vi "VIH - VI Doc Editor #2 - GenObject Properties - Write.vi"(8 "error in":errorcluster, 10 "Props":T1, 11 "Ctrl Refnum":refnum<vi>) -> (0 "error out":errorcluster, 3 "dup Ctrl Refnum":refnum<vi>)   [LabVIEW 2014]
doc: "::: VI Helpeks :::\nCopyright (c) 2000-2026 Konstantin Shifershteyn. All rights reserved."
panel:
  # "VI Helpeks\nCopyright (c) 2012-2026 Konstantin Shifershteyn"
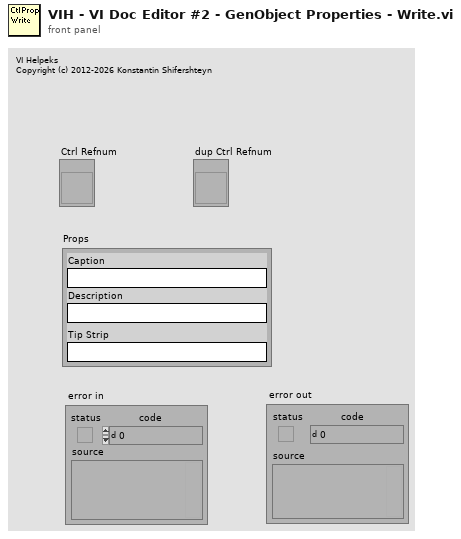
[diagram p1: front panel]
types:
  T1 = cluster{"Caption":string, "Description":string, "Tip Strip":string}
  T2 = cluster{"Has Caption":bool, "Caption":string, "Description":string, "Tip Strip":string}
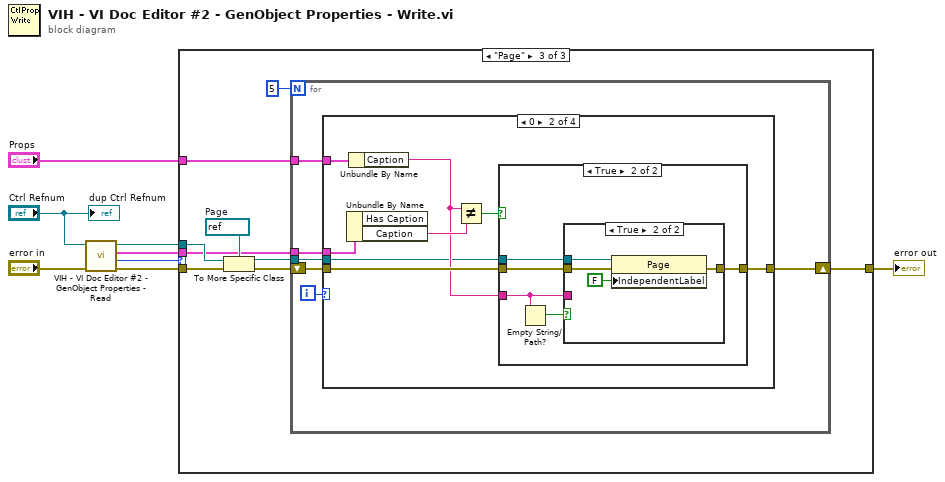
[diagram p0: block diagram]
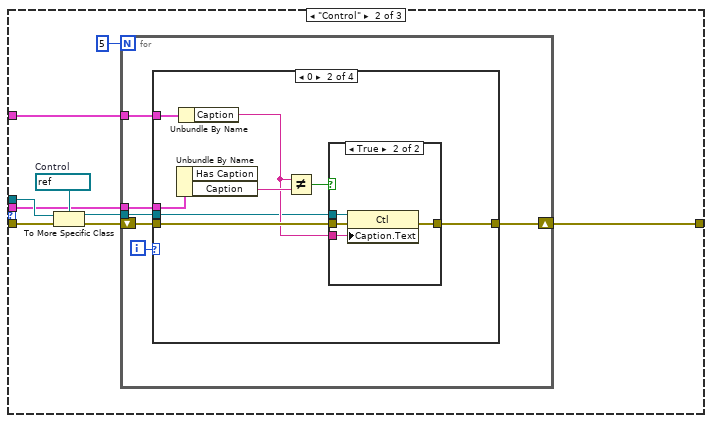
[diagram p3: hidden frame]
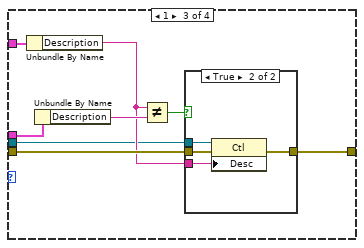
[diagram p6: hidden frame]
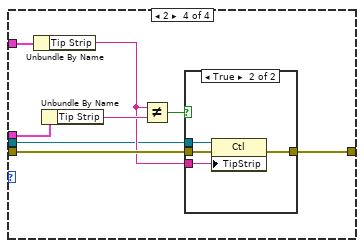
[diagram p8: hidden frame]
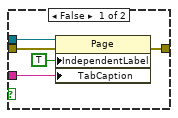
[diagram p12: hidden frame]
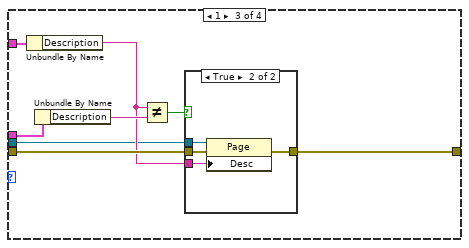
[diagram p13: hidden frame]
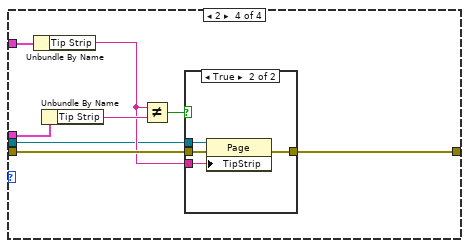
[diagram p15: hidden frame]
diagram:
  n1 = call "VIH - VI Doc Editor #2 - GenObject Properties - Read.vi"("error in"="error in", "Gen Refnum"="Ctrl Refnum") -> ("error out"=w3:errorcluster, "type"=w4:enum16{"<Invalid>", "Control", "Page"}, "Props"=w1:T2, "dup Gen Refnum"=w2:refnum<vi>)  [unwired: 6 in]
  n2 = case shown="\"Page\"" w4 {
    tunnel: "Props" -> [_ w17 w72]
    tunnel: [w9 w16 w71] -> w7
    tunnel: w3 -> [w9 w14 w69]
    tunnel: w2 -> [_ w12 w67]
    tunnel: w1 -> [_ w10 w65]
    frame "<Invalid>" {
    }
    frame "Control" {
      w15 = refnum<vi> refnum  # Control
      n3 = To More Specific Class(target class=w15, reference=w12, error in=w14) -> (specific class reference=w11:refnum<vi>, error out=w13:errorcluster)
      n4 = for {
        N: 5 -> [_]
        tunnel: w10 -> [w24]
        tunnel: w17 -> [w22]
        shift-right: [w20] -> w16
        shift-left: w13 -> [w21]
        tunnel: w11 -> [w19]
        i -> [w23]
        n5 = case shown="0" w23 {
          tunnel: w24 -> [_ w33 w46 w59]
          tunnel: w22 -> [_ w32 w45 w58]
          tunnel: w21 -> [w25 w31 w44 w57]
          tunnel: [w25 w30 w43 w56] -> w20
          tunnel: w19 -> [_ w26 w39 w52]
          frame Default {
          }
          frame 0 {
            n6 = Unbundle By Name(w33) -> ("Caption"=w29:string)  [unwired: 1 out]
            n7 = Unbundle By Name(w32) -> ("Caption"=w28:string)
            n8 = Not Equal?(x=w28, y=w29) -> (x != y?=w27:bool)
            n9 = case shown="True" w27 {
              tunnel: w31 -> [w34 w38]
              tunnel: [w34 w37] -> w30
              tunnel: w28 -> [_ w36]
              tunnel: w26 -> [_ w35]
              frame False {
              }
              frame True {
                n10 = property class="Ctl"(reference=w35, error in=w38, "Caption.Text"=w36) -> (error out=w37:errorcluster)  [unwired: 1 out]
              }
            }
          }
          frame 1 {
            n11 = Unbundle By Name(w45) -> ("Description"=w41:string)
            n12 = Unbundle By Name(w46) -> ("Description"=w42:string)
            n13 = Not Equal?(x=w41, y=w42) -> (x != y?=w40:bool)
            n14 = case shown="True" w40 {
              tunnel: w44 -> [w47 w51]
              tunnel: [w47 w50] -> w43
              tunnel: w41 -> [_ w49]
              tunnel: w39 -> [_ w48]
              frame False {
              }
              frame True {
                n15 = property class="Ctl"(reference=w48, error in=w51, "Desc"=w49) -> (error out=w50:errorcluster)  [unwired: 1 out]
              }
            }
          }
          frame 2 {
            n16 = Unbundle By Name(w58) -> ("Tip Strip"=w54:string)
            n17 = Unbundle By Name(w59) -> ("Tip Strip"=w55:string)
            n18 = Not Equal?(x=w54, y=w55) -> (x != y?=w53:bool)
            n19 = case shown="True" w53 {
              tunnel: w57 -> [w60 w64]
              tunnel: [w60 w63] -> w56
              tunnel: w54 -> [_ w62]
              tunnel: w52 -> [_ w61]
              frame False {
              }
              frame True {
                n20 = property class="Ctl"(reference=w61, error in=w64, "TipStrip"=w62) -> (error out=w63:errorcluster)  [unwired: 1 out]
              }
            }
          }
        }
      }
    }
    frame "Page" {
      w70 = refnum<vi> refnum  # Page
      n21 = To More Specific Class(target class=w70, reference=w67, error in=w69) -> (specific class reference=w66:refnum<vi>, error out=w68:errorcluster)
      n22 = for {
        N: 5 -> [_]
        tunnel: w65 -> [w79]
        tunnel: w72 -> [w77]
        shift-right: [w75] -> w71
        shift-left: w68 -> [w76]
        tunnel: w66 -> [w74]
        i -> [w78]
        n23 = case shown="0" w78 {
          tunnel: w79 -> [_ w88 w111 w124]
          tunnel: w77 -> [_ w87 w110 w123]
          tunnel: w76 -> [w80 w86 w109 w122]
          tunnel: [w80 w85 w108 w121] -> w75
          tunnel: w74 -> [_ w81 w104 w117]
          frame Default {
          }
          frame 0 {
            n24 = Unbundle By Name(w88) -> ("Caption"=w84:string)  [unwired: 1 out]
            n25 = Unbundle By Name(w87) -> ("Caption"=w83:string)
            n26 = Not Equal?(x=w83, y=w84) -> (x != y?=w82:bool)
            n27 = case shown="True" w82 {
              tunnel: w86 -> [w89 w94]
              tunnel: [w89 w93] -> w85
              tunnel: w83 -> [_ w90]
              tunnel: w81 -> [_ w92]
              frame False {
              }
              frame True {
                n28 = Empty String/Path?(string/path=w90) -> (empty?=w91:bool)
                n29 = case shown="True" w91 {
                  tunnel: w94 -> [w99 w103]
                  tunnel: [w98 w102] -> w93
                  tunnel: w92 -> [w97 w101]
                  tunnel: w90 -> [w96 _]
                  frame False {
                    n30 = property class="Page"(reference=w97, error in=w99, "IndependentLabel"=TRUE ("Independent Label"), "TabCaption"=w96) -> (error out=w98:errorcluster)  [unwired: 1 out]
                  }
                  frame True {
                    n31 = property class="Page"(reference=w101, error in=w103, "IndependentLabel"=FALSE ("Independent Label")) -> (error out=w102:errorcluster)  [unwired: 1 out]
                  }
                }
              }
            }
          }
          frame 1 {
            n32 = Unbundle By Name(w110) -> ("Description"=w106:string)
            n33 = Unbundle By Name(w111) -> ("Description"=w107:string)
            n34 = Not Equal?(x=w106, y=w107) -> (x != y?=w105:bool)
            n35 = case shown="True" w105 {
              tunnel: w109 -> [w112 w116]
              tunnel: [w112 w115] -> w108
              tunnel: w106 -> [_ w114]
              tunnel: w104 -> [_ w113]
              frame False {
              }
              frame True {
                n36 = property class="Page"(reference=w113, error in=w116, "Desc"=w114) -> (error out=w115:errorcluster)  [unwired: 1 out]
              }
            }
          }
          frame 2 {
            n37 = Unbundle By Name(w123) -> ("Tip Strip"=w119:string)
            n38 = Unbundle By Name(w124) -> ("Tip Strip"=w120:string)
            n39 = Not Equal?(x=w119, y=w120) -> (x != y?=w118:bool)
            n40 = case shown="True" w118 {
              tunnel: w122 -> [w125 w129]
              tunnel: [w125 w128] -> w121
              tunnel: w119 -> [_ w127]
              tunnel: w117 -> [_ w126]
              frame False {
              }
              frame True {
                n41 = property class="Page"(reference=w126, error in=w129, "TipStrip"=w127) -> (error out=w128:errorcluster)  [unwired: 1 out]
              }
            }
          }
        }
      }
    }
  }
  "error out" <- w7
  "dup Ctrl Refnum" <- "Ctrl Refnum"
